vi "SLSC Update Values in Tree Control.vi"(0 "Section Ref in":T3 format="%.0x", 1 "TreeControl in":refnum<vi>, 2 "Properties":string="Properties", 3 "Command Channel":string="Commands", 5 "Property tree in":string[](array[string]), 7 "NewVal":variant, 9 "SLSC Output Tree":T1(array[cluster]), 11 "error in (no error)":errorcluster, 12 "Enums":T2[](array[typedef]), 13 "Enum Strings":cluster{"name":string, string}[](array[cluster]), 14 "Modify Reset Value?":bool) -> (10 "SLSC Output Tree Out":T1(array[cluster]), 15 "error out":errorcluster)   [LabVIEW 2020, in "SLSC EDS System Explorer.lvlib"]
uses:
  SLSC EDS System Explorer.lvlib
  <vilib>/NI VeriStand/Custom Device API/Custom Device Item Ref.ctl
  SLSC EDS API/JSON parsing/enum.ctl
  <vilib>/NI VeriStand/Custom Device Tools/Custom Device Utility Library/NI VeriStand - Search for Item by Name.vi
  SLSC UI API/SLSC Tree Control.lvlib
  <vilib>/NI VeriStand/Custom Device Tools/Custom Device Utility Library/Custom Device Utility Library.lvlib
  <vilib>/NI VeriStand/Custom Device API/Custom Device API.lvlib
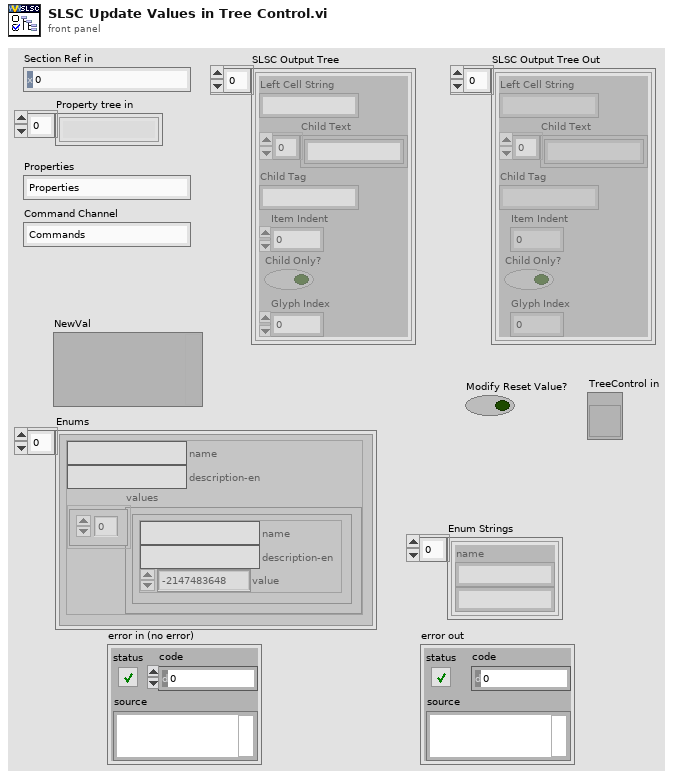
[diagram p1: front panel]
types:
  T1 = cluster{"Left Cell String":string, "Child Text":string[], "Child Tag":string, "Item Indent":i32, "Child Only?":bool, "Glyph Index":i32}[]
  T2 = typedef "enum.ctl" = cluster{"name":string, "description-en":string, "values":cluster{"name":string, "description-en":string, "value":i32}[]}
  T3 = typedef "Custom Device API.lvlib/Custom Device Item Ref.ctl" = u64
  T4 = cluster{"Left Cell String":string, "Child Text":string[], "Child Tag":string, "Item Indent":i32, "Child Only?":bool, "Glyph Index":i32}
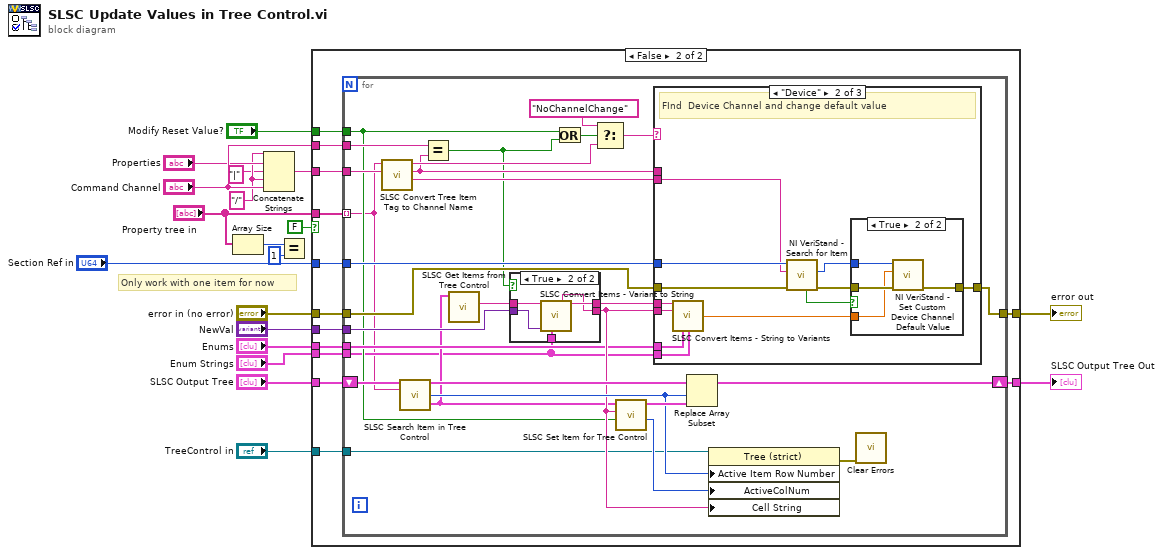
[diagram p0: block diagram]
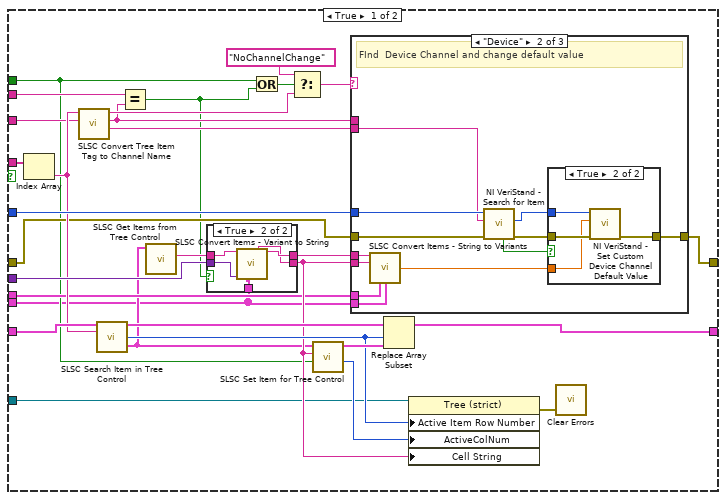
[diagram p2: hidden frame]
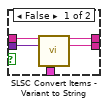
[diagram p3: hidden frame]
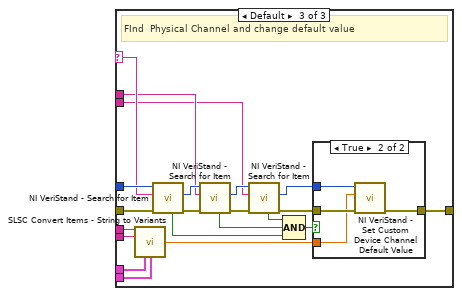
[diagram p6: hidden frame]
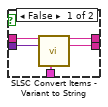
[diagram p8: hidden frame]
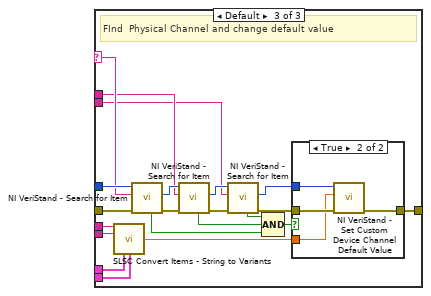
[diagram p11: hidden frame]
diagram:
  w14 = "/" ("string")
  # "Only work with one item for now"
  n1 = Array Size(array="Property tree in") -> (size(s)=w4:i32)
  n2 = Concatenate Strings(w14, "Properties", "|" ("string"), w14, "Command Channel") -> (w16:string)
  n3 = Equal?(x=w4, y=1) -> ()  [unwired: 1 out]
  n4 = case shown="False" FALSE {
    tunnel: "Section Ref in" -> [w42 w113]
    tunnel: "SLSC Output Tree" -> [w49 w116]
    tunnel: "Enums" -> [w35 w110]
    tunnel: "NewVal" -> [w44 w114]
    tunnel: "Property tree in" -> [w48 w104]
    tunnel: [w45 w115] -> w12
    tunnel: "Enum Strings" -> [w21 w105]
    tunnel: "error in (no error)" -> [w37 w112]
    tunnel: [w36 w111] -> w11
    tunnel: w16 -> [w28 w109]
    tunnel: "Command Channel" -> [w27 w108]
    tunnel: "Modify Reset Value?" -> [w25 w107]
    tunnel: "TreeControl in" -> [w24 w106]
    frame True {
      n5 = Index Array(array=w48) -> (element=w41:string)  [unwired: 1 in]
      n6 = call "SLSC Convert Tree Item Tag to Channel Name.vi"("Type of Item"=w28, "Item String"=w41) -> ("Item Name"=w40:string, "Type of Item"=w29:string, "Device/Physical Channel"=w30:string)  [unwired: 7 in]
      n7 = call "SLSC Search Item in Tree Control.vi"("SLSC Output Tree"=w49, "Item Tag"=w41) -> ("SLSC Output Tree Out"=w47:T1, "Position"=w43:i32, "Item"=w34:T4)  [unwired: 10 in, 1 out]
      n8 = Equal?(x=w27, y=w29) -> (x = y?=w20:bool)
      n9 = call "SLSC Get Items from Tree Control.vi"("Item"=w34) -> ("Datatype"=w22:string)  [unwired: 6 in, 4 out]
      n10 = case shown="True" w20 {
        tunnel: w44 -> [w54 w56]
        tunnel: [w53 w55] -> w39
        tunnel: [w52 w59] -> w38
        tunnel: w22 -> [w51 w58]
        tunnel: w21 -> [w50 w57]
        frame False {
          n11 = call "SLSC Convert Items - Variant to String.vi"("Datatype"=w51, "value"=w54, "Enum string"=w50) -> ("Output data type"=w52:string, "string data value"=w53:string)  [unwired: 6 in, 5 out]
        }
        frame True {
          n12 = call "SLSC Convert Items - Variant to String.vi"("Datatype"=w58, "reset value"=w56, "Enum string"=w57) -> ("string data reset value"=w55:string, "Output data type"=w59:string)  [unwired: 6 in, 5 out]
        }
      }
      n13 = Or(x=w25, y=w20) -> (x .or. y?=w26:bool)
      n14 = Select(t="NoChannelChange", s=w26, f=w30) -> (s? t:f=w33:string)
      n15 = call "SLSC Set Item for Tree Control.vi"("Modify Reset Value?"=w25, "Value"=w39, "Item In"=w34) -> ("Changed Column"=w31:i32, "Item Out"=w46:T4)  [unwired: 7 in]
      n16 = case shown="\"Device\"" w33 {
        selector: w33 -> [_ _ w95]
        tunnel: w42 -> [_ w72 w98]
        tunnel: w40 -> [_ w71 w88]
        tunnel: w39 -> [_ w64 w85]
        tunnel: w38 -> [_ w65 w86]
        tunnel: w37 -> [w60 w68 w97]
        tunnel: [w60 w66 w96] -> w36
        tunnel: w21 -> [_ w62 w83]
        tunnel: w35 -> [_ w63 w84]
        tunnel: w29 -> [_ _ w89]
        frame "NoChannelChange" {
          # "Do nothing"
        }
        frame "Device" {
          # "FInd  Device Channel and change default value"
          n17 = call "SLSC Convert Items - String to Variants.vi"("Datatype"=w65, "Value"=w64, "enums"=w63, "string enums"=w62) -> ("Value (DBL)"=w61:dbl)  [unwired: 8 in, 3 out]
          n18 = call-poly <vilib>:"NI VeriStand - Search for Item.vi"("error in"=w68, "Item Name"=w71, "Section Ref in"=w72) -> ("error out"=w67:errorcluster, "Item Ref"=w69:T3, "Found"=w70:bool)  [unwired: 5 in, 1 out]
          n19 = case shown="True" w70 {
            tunnel: w69 -> [_ w77]
            tunnel: w67 -> [w73 w76]
            tunnel: [w73 w75] -> w66
            tunnel: w61 -> [_ w74]
            frame False {
            }
            frame True {
              n20 = call <vilib>:"NI VeriStand - Set Custom Device Channel Default Value.vi"("error in (no error)"=w76, "Default Value"=w74, "Channel Ref in"=w77) -> ("error out"=w75:errorcluster)  [unwired: 7 in, 1 out]
            }
          }
        }
        frame Default {
          # "FInd  Physical Channel and change default value"
          n21 = call "SLSC Convert Items - String to Variants.vi"("Datatype"=w86, "Value"=w85, "enums"=w84, "string enums"=w83) -> ("Value (DBL)"=w82:dbl)  [unwired: 8 in, 3 out]
          n22 = call-poly <vilib>:"NI VeriStand - Search for Item.vi"("error in"=w97, "Item Name"=w95, "Section Ref in"=w98) -> ("error out"=w94:errorcluster, "Item Ref"=w93:T3, "Found"=w78:bool)  [unwired: 5 in, 1 out]
          n23 = call-poly <vilib>:"NI VeriStand - Search for Item.vi"("error in"=w94, "Item Name"=w89, "Section Ref in"=w93) -> ("error out"=w92:errorcluster, "Item Ref"=w91:T3, "Found"=w79:bool)  [unwired: 5 in, 1 out]
          n24 = call-poly <vilib>:"NI VeriStand - Search for Item.vi"("error in"=w92, "Item Name"=w88, "Section Ref in"=w91) -> ("error out"=w87:errorcluster, "Item Ref"=w90:T3, "Found"=w80:bool)  [unwired: 5 in, 1 out]
          n25 = Compound Arithmetic op=AND(w80, w79, w78) -> (w81:bool)
          n26 = case shown="True" w81 {
            tunnel: w90 -> [_ w103]
            tunnel: w87 -> [w99 w102]
            tunnel: [w99 w101] -> w96
            tunnel: w82 -> [_ w100]
            frame False {
            }
            frame True {
              n27 = call <vilib>:"NI VeriStand - Set Custom Device Channel Default Value.vi"("error in (no error)"=w102, "Default Value"=w100, "Channel Ref in"=w103) -> ("error out"=w101:errorcluster)  [unwired: 7 in, 1 out]
            }
          }
        }
      }
      n28 = Replace Array Subset(array=w47, new element=w46, index=w43) -> (w45:T1)
      n29 = property class="Tree (strict)"(reference=w24, "Active Item Row Number"=w43, "ActiveColNum"=w31, "Cell String"=w39) -> (error out=w23:errorcluster)  [unwired: 1 in, 1 out]
      n30 = call <vilib>:"Clear Errors.vi"("error in (no error)"=w23) -> ()  [unwired: 5 in, 2 out]
    }
    frame False {
      n31 = for {
        tunnel: w114 -> [w141]
        tunnel: w113 -> [w139]
        tunnel: w110 -> [w133]
        tunnel: w109 -> [w126]
        tunnel: w108 -> [w125]
        tunnel: w107 -> [w123]
        tunnel: w106 -> [w122]
        tunnel: w105 -> [w119]
        shift-right: [w142] -> w115
        shift-left: w116 -> [w145]
        tunnel: w104 -> [w117] mode=indexing
        tunnel: w112 -> [w135]
        tunnel: [w134] -> w111
        n32 = call "SLSC Convert Tree Item Tag to Channel Name.vi"("Type of Item"=w126, "Item String"=w117) -> ("Item Name"=w138:string, "Type of Item"=w127:string, "Device/Physical Channel"=w128:string)  [unwired: 7 in]
        n33 = call "SLSC Search Item in Tree Control.vi"("SLSC Output Tree"=w145, "Item Tag"=w117) -> ("SLSC Output Tree Out"=w144:T1, "Position"=w140:i32, "Item"=w132:T4)  [unwired: 10 in, 1 out]
        n34 = Equal?(x=w125, y=w127) -> (x = y?=w118:bool)
        n35 = call "SLSC Get Items from Tree Control.vi"("Item"=w132) -> ("Datatype"=w120:string)  [unwired: 6 in, 4 out]
        n36 = case shown="True" w118 {
          tunnel: w141 -> [w150 w152]
          tunnel: [w149 w151] -> w137
          tunnel: [w148 w155] -> w136
          tunnel: w120 -> [w147 w154]
          tunnel: w119 -> [w146 w153]
          frame False {
            n37 = call "SLSC Convert Items - Variant to String.vi"("Datatype"=w147, "value"=w150, "Enum string"=w146) -> ("Output data type"=w148:string, "string data value"=w149:string)  [unwired: 6 in, 5 out]
          }
          frame True {
            n38 = call "SLSC Convert Items - Variant to String.vi"("Datatype"=w154, "reset value"=w152, "Enum string"=w153) -> ("string data reset value"=w151:string, "Output data type"=w155:string)  [unwired: 6 in, 5 out]
          }
        }
        n39 = Or(x=w123, y=w118) -> (x .or. y?=w124:bool)
        n40 = Select(t="NoChannelChange", s=w124, f=w128) -> (s? t:f=w131:string)
        n41 = call "SLSC Set Item for Tree Control.vi"("Modify Reset Value?"=w123, "Value"=w137, "Item In"=w132) -> ("Changed Column"=w129:i32, "Item Out"=w143:T4)  [unwired: 7 in]
        n42 = case shown="\"Device\"" w131 {
          selector: w131 -> [_ _ w191]
          tunnel: w139 -> [_ w168 w194]
          tunnel: w138 -> [_ w167 w184]
          tunnel: w137 -> [_ w160 w181]
          tunnel: w136 -> [_ w161 w182]
          tunnel: w135 -> [w156 w164 w193]
          tunnel: [w156 w162 w192] -> w134
          tunnel: w119 -> [_ w158 w179]
          tunnel: w133 -> [_ w159 w180]
          tunnel: w127 -> [_ _ w185]
          frame "NoChannelChange" {
            # "Do nothing"
          }
          frame "Device" {
            # "FInd  Device Channel and change default value"
            n43 = call "SLSC Convert Items - String to Variants.vi"("Datatype"=w161, "Value"=w160, "enums"=w159, "string enums"=w158) -> ("Value (DBL)"=w157:dbl)  [unwired: 8 in, 3 out]
            n44 = call-poly <vilib>:"NI VeriStand - Search for Item.vi"("error in"=w164, "Item Name"=w167, "Section Ref in"=w168) -> ("error out"=w163:errorcluster, "Item Ref"=w165:T3, "Found"=w166:bool)  [unwired: 5 in, 1 out]
            n45 = case shown="True" w166 {
              tunnel: w165 -> [_ w173]
              tunnel: w163 -> [w169 w172]
              tunnel: [w169 w171] -> w162
              tunnel: w157 -> [_ w170]
              frame False {
              }
              frame True {
                n46 = call <vilib>:"NI VeriStand - Set Custom Device Channel Default Value.vi"("error in (no error)"=w172, "Default Value"=w170, "Channel Ref in"=w173) -> ("error out"=w171:errorcluster)  [unwired: 7 in, 1 out]
              }
            }
          }
          frame Default {
            # "FInd  Physical Channel and change default value"
            n47 = call "SLSC Convert Items - String to Variants.vi"("Datatype"=w182, "Value"=w181, "enums"=w180, "string enums"=w179) -> ("Value (DBL)"=w178:dbl)  [unwired: 8 in, 3 out]
            n48 = call-poly <vilib>:"NI VeriStand - Search for Item.vi"("error in"=w193, "Item Name"=w191, "Section Ref in"=w194) -> ("error out"=w190:errorcluster, "Item Ref"=w189:T3, "Found"=w174:bool)  [unwired: 5 in, 1 out]
            n49 = call-poly <vilib>:"NI VeriStand - Search for Item.vi"("error in"=w190, "Item Name"=w185, "Section Ref in"=w189) -> ("error out"=w188:errorcluster, "Item Ref"=w187:T3, "Found"=w175:bool)  [unwired: 5 in, 1 out]
            n50 = call-poly <vilib>:"NI VeriStand - Search for Item.vi"("error in"=w188, "Item Name"=w184, "Section Ref in"=w187) -> ("error out"=w183:errorcluster, "Item Ref"=w186:T3, "Found"=w176:bool)  [unwired: 5 in, 1 out]
            n51 = Compound Arithmetic op=AND(w176, w175, w174) -> (w177:bool)
            n52 = case shown="True" w177 {
              tunnel: w186 -> [_ w199]
              tunnel: w183 -> [w195 w198]
              tunnel: [w195 w197] -> w192
              tunnel: w178 -> [_ w196]
              frame False {
              }
              frame True {
                n53 = call <vilib>:"NI VeriStand - Set Custom Device Channel Default Value.vi"("error in (no error)"=w198, "Default Value"=w196, "Channel Ref in"=w199) -> ("error out"=w197:errorcluster)  [unwired: 7 in, 1 out]
              }
            }
          }
        }
        n54 = Replace Array Subset(array=w144, new element=w143, index=w140) -> (w142:T1)
        n55 = property class="Tree (strict)"(reference=w122, "Active Item Row Number"=w140, "ActiveColNum"=w129, "Cell String"=w137) -> (error out=w121:errorcluster)  [unwired: 1 in, 1 out]
        n56 = call <vilib>:"Clear Errors.vi"("error in (no error)"=w121) -> ()  [unwired: 5 in, 2 out]
      }
    }
  }
  "SLSC Output Tree Out" <- w12
  "error out" <- w11
